vi "AWS_Sequence_Load_data.vi"(8 "error in":errorcluster, 11 "appended path":path) -> (0 "error out":errorcluster, 3 "S array":T3(array[cluster]))   [LabVIEW 2018]
panel:
  out "Base Table":T1(array[cluster])
  out "data":string[][](array[string])
  out "STD Type":enum16{"Region", "Each", "Fixed"}(ring)
  out "S New Info and MiN out":T2={"Sample Sequence"="GATGATGATGATGATGAT", "Right Read MIN"=6, "Filter P"=0, "STD Type"=enum."Region", "Base Table"=[], "Selection"=enum."10kHz", "noise MAX"=3, "Sample name"=""} {"Base Table"."Value 3" format="%.2g"}
  out "Selection":enum16{"10kHz", "100kHz"}(ring)
  out "SQ_Table_array":string[][](array[string])
  out "channel names":string[](array[string])
  out "group names":string[](array[string])
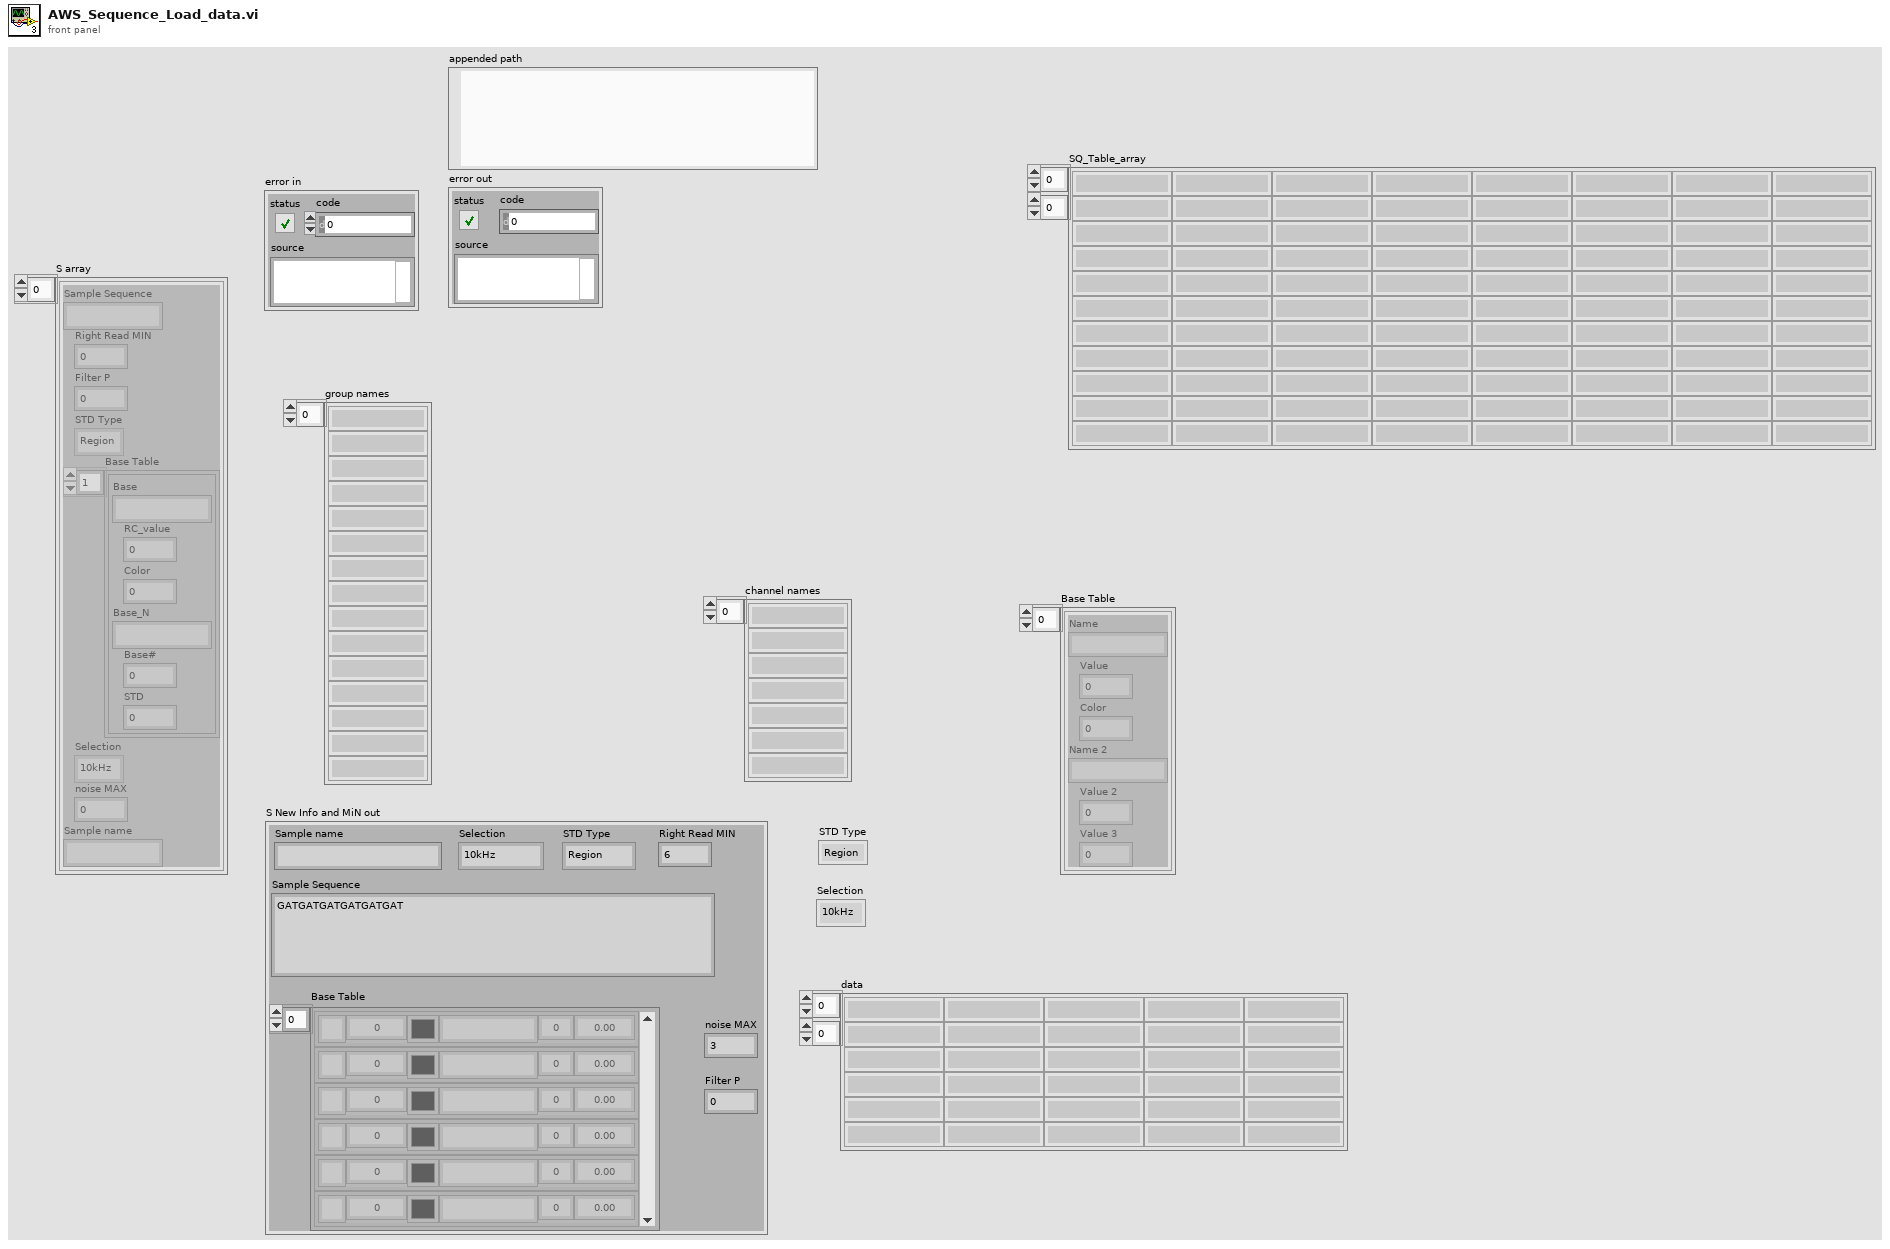
[diagram p1: front panel]
types:
  T1 = cluster{"Name":string, "Value":dbl, "Color":u32, "Name 2":string, "Value 2":dbl, "Value 3":dbl}[]
  T2 = cluster{"Sample Sequence":string, "Right Read MIN":i32, "Filter P":i32, "STD Type":enum16{"Region", "Each", "Fixed"}, "Base Table":cluster{"Name":string, "Value":dbl, "Color":u32, "Name 2":string, "Value 2":dbl, "Value 3":dbl}[], "Selection":enum16{"10kHz", "100kHz"}, "noise MAX":i32, "Sample name":string}
  T3 = cluster{"Sample Sequence":string, "Right Read MIN":i32, "Filter P":i32, "STD Type":enum16{"Region", "Each", "Fixed"}, "Base Table":cluster{"Base":string, "RC_value":dbl, "Color":u32, "Base_N":string, "Base#":dbl, "STD":dbl}[], "Selection":enum16{"10kHz", "100kHz"}, "noise MAX":i32, "Sample name":string}[]
  T4 = cluster{"group name":string, dbl, i32, "group name":string, dbl, dbl}
  T5 = cluster{"group name":string, i32, i32, i32, cluster{"group name":string, dbl, i32, "group name":string, dbl, dbl}[], i32, i32, "group name":string}
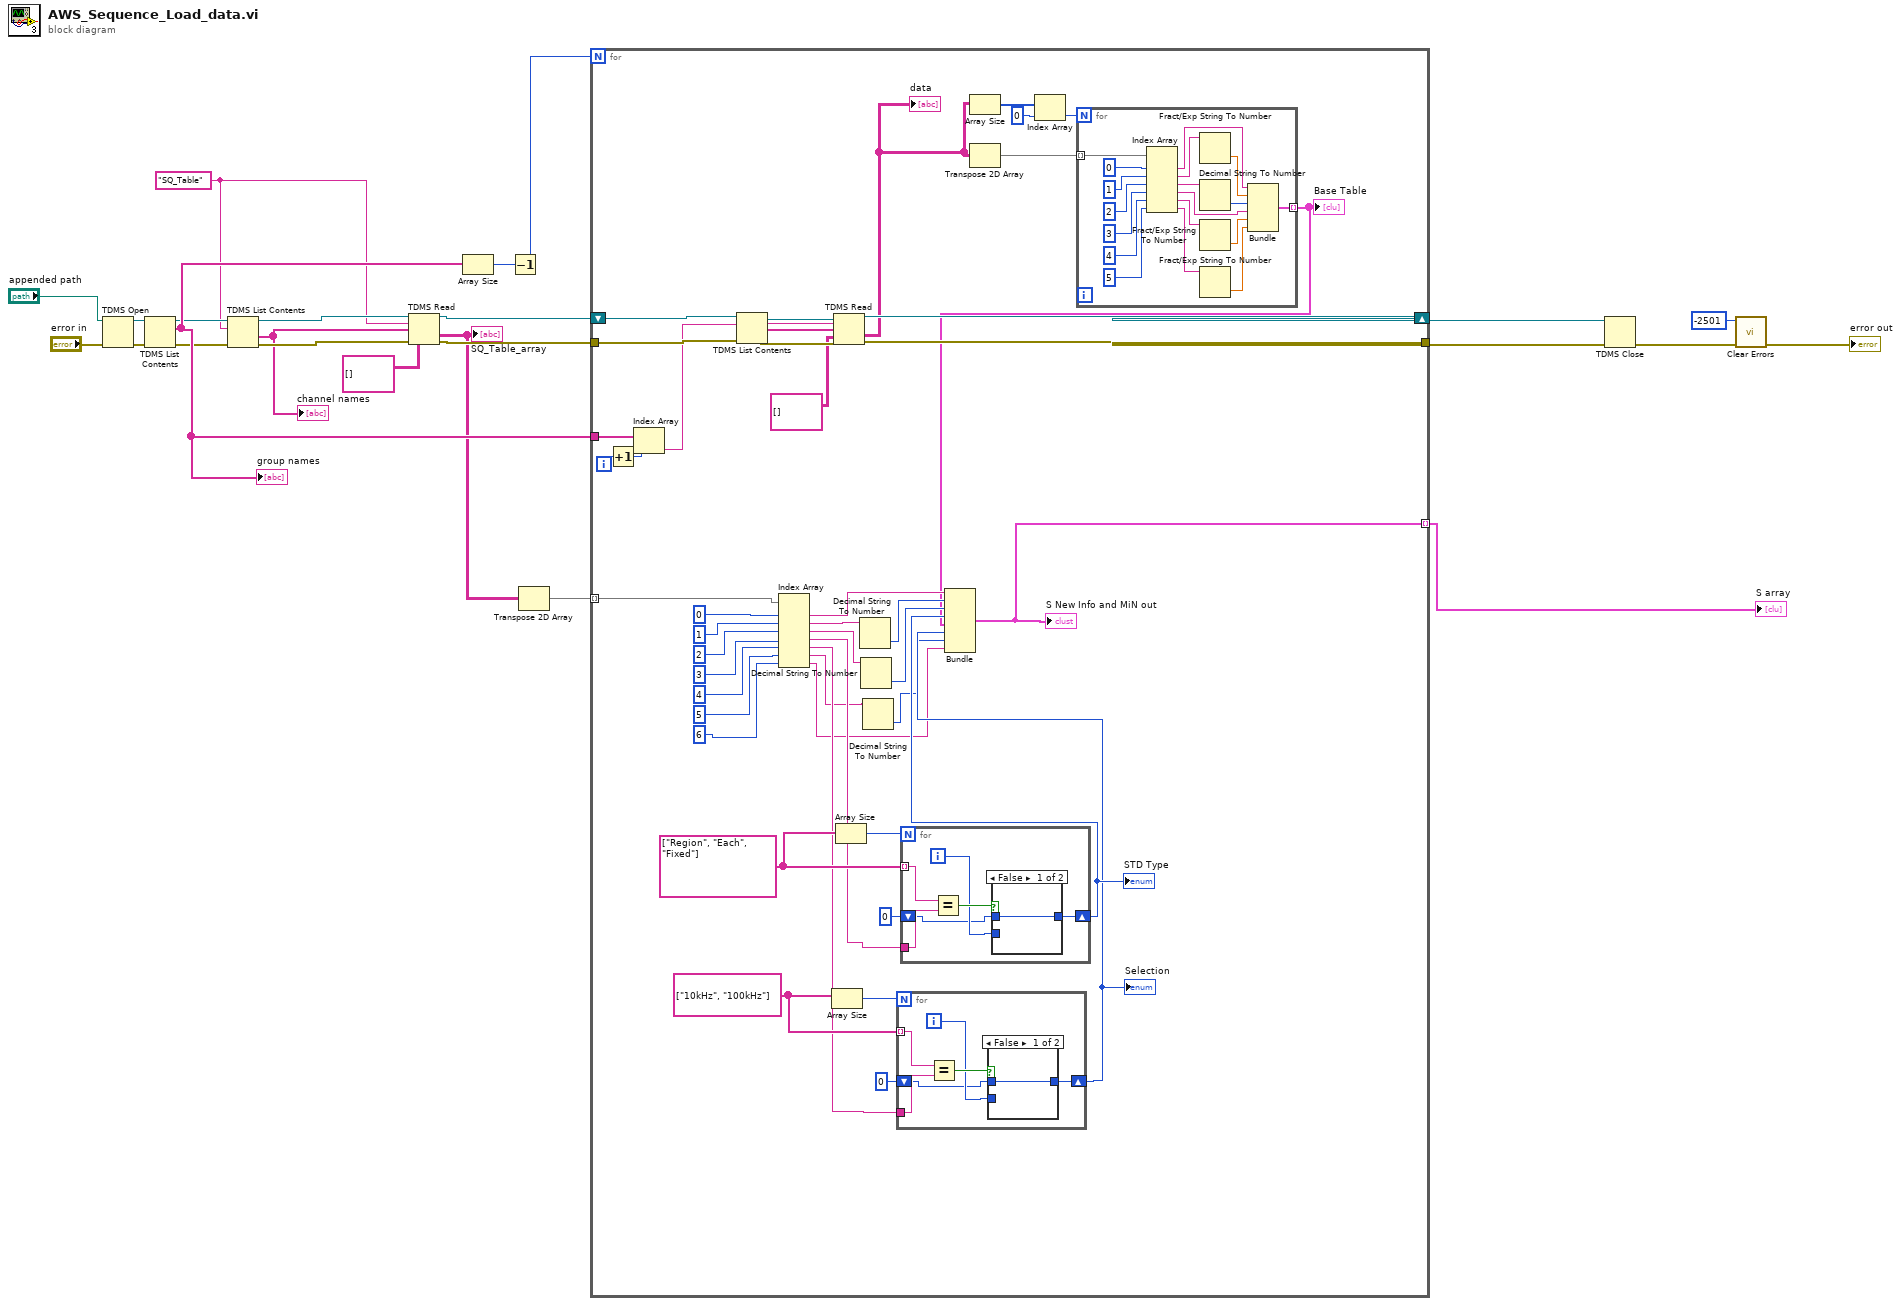
[diagram p0: block diagram]
diagram:
  w9 = "SQ_Table" ("group name in")
  n1 = TDMS Open(8:"error in", 11:"appended path") -> (0:w21:errorcluster, 3:w20:refnum<k34>)  [unwired: 5 in]
  n2 = TDMS List Contents(4:w21, 7:w20) -> (0:w13:errorcluster, 2:w16:string[], 3:w11:refnum<k34>)  [unwired: 1 in, 1 out]
  "group names" <- w16
  n3 = TDMS List Contents(4:w13, 6:w9, 7:w11) -> (0:w12:errorcluster, 1:w8:string[], 3:w10:refnum<k34>)  [unwired: 1 out]
  "channel names" <- w8
  n4 = TDMS Read(0:w10, 5:w9, 7:w8, 11:w12, 12:string[][] [] ("group name")) -> (4:w14:refnum<k34>, 10:w3:string[][], 15:w15:errorcluster)  [unwired: 3 in, 3 out]
  "SQ_Table_array" <- w3
  n5 = Array Size(array=w16) -> (size(s)=w17:i32)
  n6 = Decrement(x=w17) -> (x-1=w4:i32)
  n7 = Transpose 2D Array(2D array=w3) -> (transposed array=w2:string[][])
  n8 = for {
    N: w4 -> [_]
    shift-right: [w69] -> w19
    shift-left: w14 -> [w68]
    tunnel: w15 -> [w66]
    tunnel: [w70] -> w18
    tunnel: w16 -> [w61]
    tunnel: w2 -> [w58] mode=indexing
    tunnel: [w26] -> w1 mode=indexing
    i -> [w60]
    w47 = string[] ["10kHz", "100kHz"] ("Strings []")
    w45 = string[] ["Region", "Each", "Fixed"] ("STD []")
    n9 = Increment(x=w60) -> (x+1=w25:i32)
    n10 = Index Array(array=w61, index=w25) -> (element=w59:string)
    n11 = TDMS List Contents(4:w66, 6:w59, 7:w68) -> (0:w65:errorcluster, 1:w64:string[], 2:w62:string, 3:w67:refnum<k34>)
    n12 = Index Array(array=w58, index #1=0 ("index"), index #2=1 ("index"), index #3=2 ("index"), index #4=3 ("index"), index #5=4 ("index"), index #6=5 ("index"), index #7=6 ("index")) -> (element #1=w56:string, element #2=w54:string, element #3=w51:string, element #4=w42:string, element #5=w41:string, element #6=w36:string, element #7=w33:string)
    n13 = Array Size(array=w47) -> (size(s)=w49:i32)
    n14 = TDMS Read(0:w67, 5:w62, 7:w64, 11:w65, 12:string[][] [] ("group name")) -> (4:w69:refnum<k34>, 10:w28:string[][], 15:w70:errorcluster)  [unwired: 3 in, 3 out]
    "data" <- w28
    n15 = Array Size(array=w45) -> (size(s)=w48:i32)
    n16 = Decimal String To Number(string=w54) -> (number=w53:i32)  [unwired: 2 in, 1 out]
    n17 = Decimal String To Number(string=w51) -> (number=w50:i32)  [unwired: 2 in, 1 out]
    n18 = Decimal String To Number(string=w36) -> (number=w35:i32)  [unwired: 2 in, 1 out]
    n19 = for {
      N: w49 -> [_]
      tunnel: w47 -> [w94] mode=indexing
      tunnel: w41 -> [w93]
      shift-right: [w90] -> w38
      shift-left: 0 -> [w89]
      i -> [w91]
      n20 = Equal?(x=w94, y=w93) -> (x = y?=w92:bool)
      n21 = case shown="False" w92 {
        tunnel: w91 -> [_ w96]
        tunnel: [w95 w96] -> w90
        tunnel: w89 -> [w95 _]
        frame False {
        }
        frame True {
        }
      }
    }
    "Selection" <- w38
    n22 = for {
      N: w48 -> [_]
      tunnel: w45 -> [w102] mode=indexing
      tunnel: w42 -> [w101]
      shift-right: [w98] -> w39
      shift-left: 0 -> [w97]
      i -> [w99]
      n23 = Equal?(x=w102, y=w101) -> (x = y?=w100:bool)
      n24 = case shown="False" w100 {
        tunnel: w99 -> [_ w104]
        tunnel: [w103 w104] -> w98
        tunnel: w97 -> [w103 _]
        frame False {
        }
        frame True {
        }
      }
    }
    "STD Type" <- w39
    n25 = Array Size(array=w28) -> (size(s)=w32:i32[])
    n26 = Transpose 2D Array(2D array=w28) -> (transposed array=w29:string[][])
    n27 = Index Array(array=w32, index=0) -> (element=w30:i32)
    n28 = for {
      N: w30 -> [_]
      tunnel: w29 -> [w88] mode=indexing
      tunnel: [w71] -> w27 mode=indexing
      n29 = Index Array(array=w88, index #1=0 ("index"), index #2=1 ("index"), index #3=2 ("index"), index #4=3 ("index"), index #5=4 ("index"), index #6=5 ("index")) -> (element #1=w81:string, element #2=w79:string, element #3=w77:string, element #4=w80:string, element #5=w75:string, element #6=w74:string)
      n30 = Fract/Exp String To Number(string=w79) -> (number=w78:dbl)  [unwired: 3 in, 1 out]
      n31 = Decimal String To Number(string=w77) -> (number=w76:i32)  [unwired: 2 in, 1 out]
      n32 = Fract/Exp String To Number(string=w75) -> (number=w73:dbl)  [unwired: 3 in, 1 out]
      n33 = Fract/Exp String To Number(string=w74) -> (number=w72:dbl)  [unwired: 3 in, 1 out]
      n34 = Bundle("group name"=w81, w78, w76, "group name"=w80, w73, w72) -> (w71:T4)  [unwired: 1 in]
    }
    "Base Table" <- w27
    n35 = Bundle("group name"=w56, w53, w50, w39, w27, w38, w35, "group name"=w33) -> (w26:T5)  [unwired: 1 in]
    "S New Info and MiN out" <- w26
  }
  "S array" <- w1
  n36 = TDMS Close(8:w18, 11:w19) -> (0:w22:errorcluster)  [unwired: 1 out]
  n37 = call <vilib>:"Clear Errors.vi"("error in (no error)"=w22, "specific error code to clear (0: all)"=-2501) -> ("error out"=→"error out":errorcluster)  [unwired: 4 in, 1 out]
